vi "Example_Simple.vi"() -> ()   [LabVIEW 2019]
doc: "- - -\nCopyright (c) 2026, Merecs Engineering GmbH"
uses:
  Language Selection/Language Selection.lvlib
panel:
  in  "Tab Control":enum32{"Page 1", "Page 2", "INFO EDITOR"}(tab)
  out "Simple_String":string caption="String"
  out "Constant String":string caption="Constant"
  in  "Quit":bool caption="stop"
  in  "Select Language":string(combo) caption="Language"
  # "Info: Unicode in tabs How-To will be added later"
  # "Info: More controls will be added later"
  # "To edit the language file start the Language Editor from the LabVIEW menu\n*Tools » Merecs Engineering » Merecs Language Toolkit » Language Editor...*\n\nSelect the following paths"
  # "C:\\Program Files\\National Instruments\\LabVIEW 2019\\examples\\Merecs Engineering\\Merecs Language Toolkit"
  # "C:\\Program Files\\National Instruments\\LabVIEW 2019\\examples\\Merecs Engineering\\Merecs Language Toolkit\\Examples\\Simple_Translations.json"
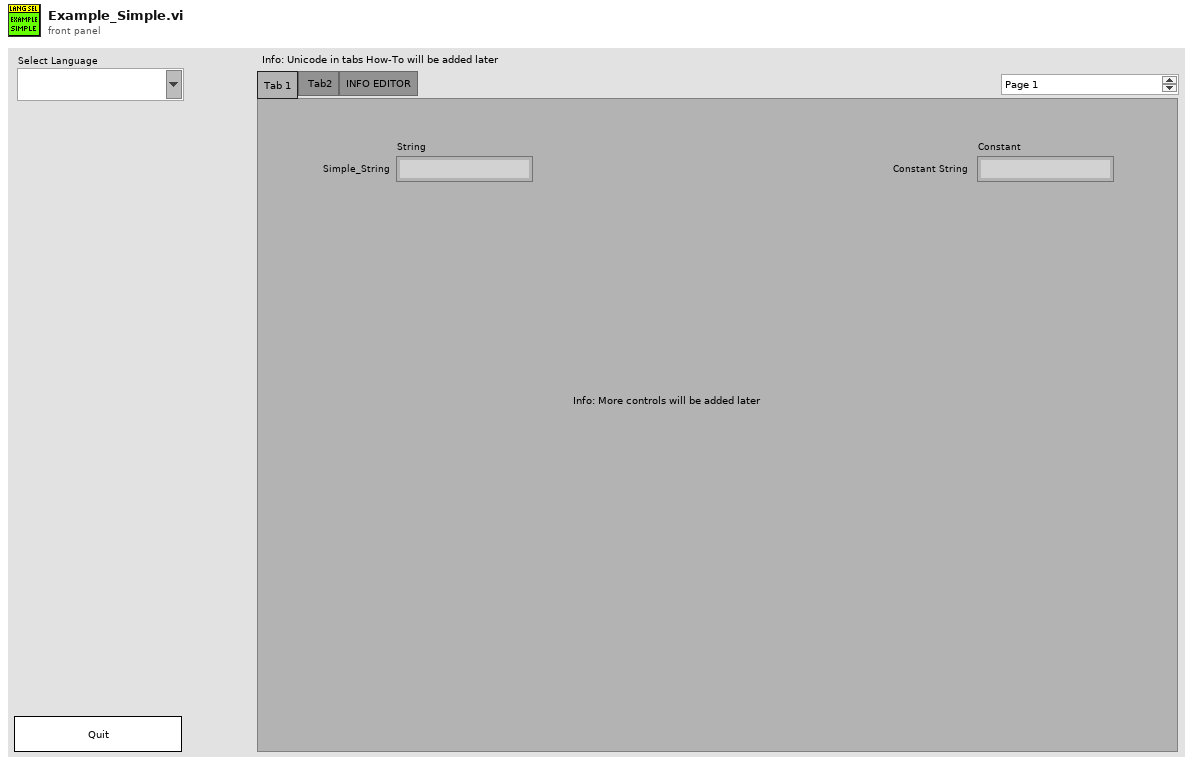
[diagram p1: front panel]
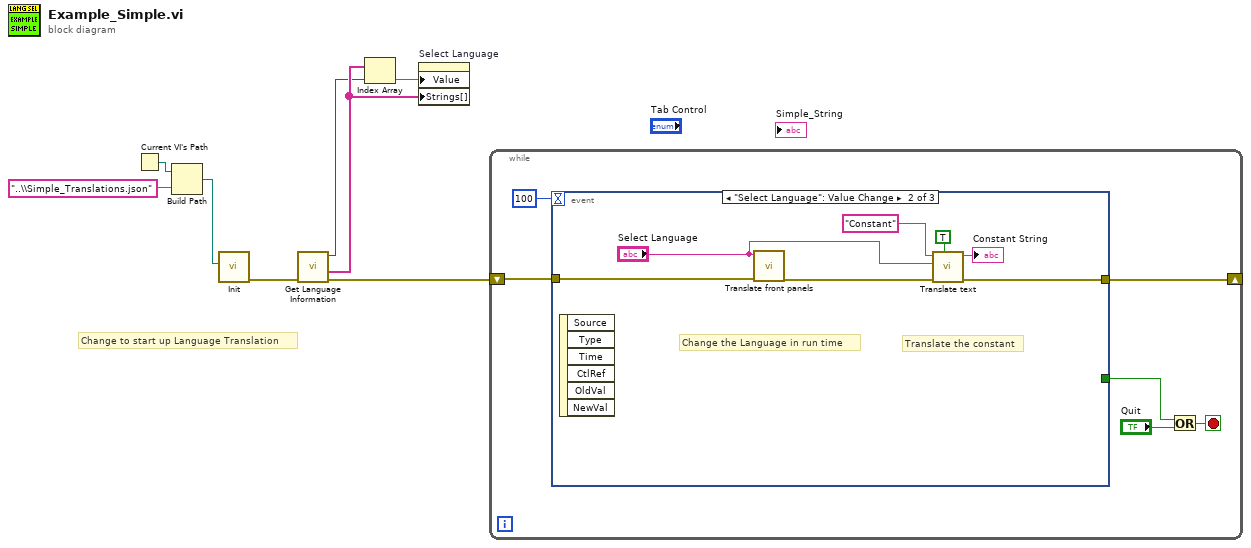
[diagram p0: block diagram]
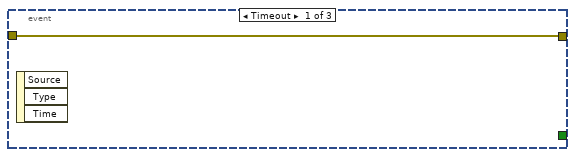
[diagram p2: hidden frame]
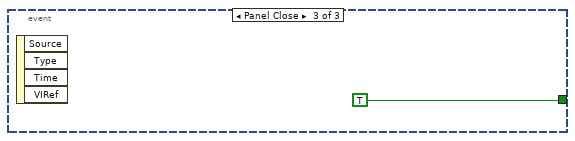
[diagram p3: hidden frame]
diagram:
  # "Change to start up Language Translation"
  n1 = Current VI's Path() -> (path=w6:path)
  n2 = Build Path(base path=w6, name or relative path="..\\Simple_Translations.json") -> (appended path=w4:path)
  n3 = call "Init.vi"("Language Translation file"=w4) -> ("error out"=w8:errorcluster)  [unwired: 9 in, 1 out]
  n4 = call "Get Language Information.vi"("error in (no error)"=w8) -> ("error out"=w7:errorcluster, "Languages"=w3:string[], "Start up Language"=w1:i32)  [unwired: 7 in, 1 out]
  n5 = Index Array(array=w3, index=w1) -> (element=w2:string)
  n6 = property on="Select Language" class="CmbBox"("Value"=w2, "Strings[]"=w3) -> ()  [unwired: 2 in, 2 out]
  n7 = while {
    shift-right: [w11] -> _
    shift-left: w7 -> [w12]
    stop <- w10 stop-if-true
    n8 = event shown="[1] \"Select Language\": Value Change" {
      selector: _ -> [_ _ _]
      dyn-events: _ -> [_ _ _]
      timeout: 100 -> [_ _ _]
      tunnel: w12 -> [w15 w17 _]
      tunnel: [w15 w16 _] -> w11
      tunnel: [_ _ TRUE] -> w9
      event Timeout {
        n9 = event-data() -> ()  [unwired: 1 in, 3 out]
      }
      event "Select Language": Value Change {
        # "Translate the constant"
        # "Change the Language in run time"
        n10 = event-data() -> ()  [unwired: 1 in, 6 out]
        n11 = call "Translate front panels.vi"("error in (no error)"=w17, "Language"="Select Language") -> ("error out"=w20:errorcluster)  [unwired: 8 in]
        n12 = call "Translate text.vi"("Translate? (T)"=TRUE ("Translate?"), "error in (no error)"=w20, "Language(\"\"=Startup Language)"="Select Language", "Constant"="Constant" ("String")) -> ("error out"=w16:errorcluster, "Output"=→"Constant String":string)  [unwired: 6 in]
      }
      event Panel Close {
        n13 = event-data() -> ()  [unwired: 1 in, 4 out]
      }
    }
    n14 = Or(x=w9, y="Quit") -> (x .or. y?=w10:bool)
  }
